vi "Read VISA resource name.vi"(8 "error in (no error)":errorcluster, 11 "AUDIX EM1000 in":refnum<class "AUDIX EM1000.lvclass">) -> (0 "error out":errorcluster, 2 "VISA resource name":refnum<visa-resource-name>, 3 "AUDIX EM1000 out":refnum<class "AUDIX EM1000.lvclass">)   [LabVIEW 2023, in "Turn Table and Mast.lvlib" / "AUDIX EM1000.lvclass"]
uses:
  AUDIX EM1000.lvclass
  AUDIX EM1000.lvclass/AUDIX EM1000.ctl
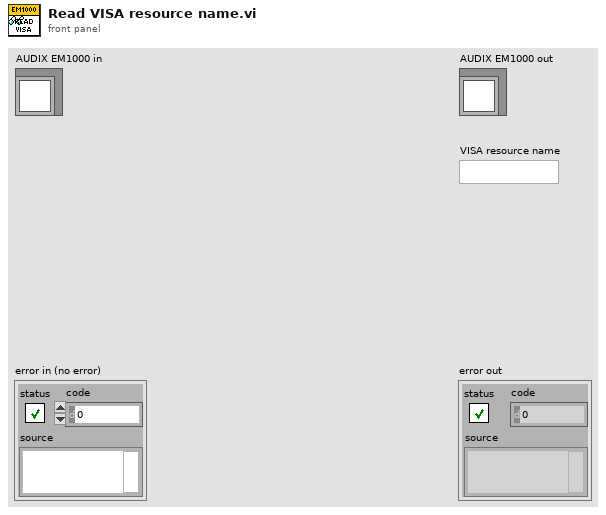
[diagram p1: front panel]
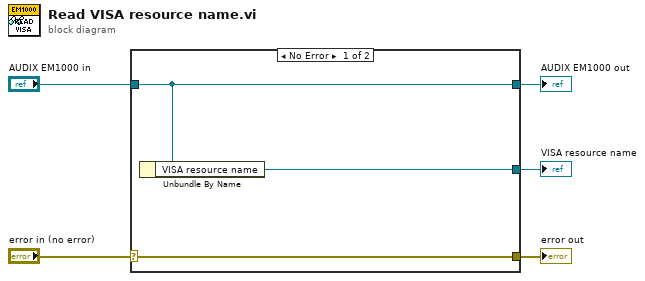
[diagram p0: block diagram]
diagram:
  n1 = case shown="No Error" "error in (no error)" {
    selector: "error in (no error)" -> [w8 w9]
    tunnel: [w8 w9] -> w4
    tunnel: [w7 w10] -> w2
    tunnel: "AUDIX EM1000 in" -> [w7 w10]
    tunnel: [w6 _] -> w1
    frame No Error {
      n2 = Unbundle By Name(w7) -> ("VISA resource name"=w6:refnum<visa-resource-name>)
    }
    frame Error {
    }
  }
  "error out" <- w4
  "AUDIX EM1000 out" <- w2
  "VISA resource name" <- w1
